vi "beepstatus.vi"() -> ()   [LabVIEW 2026]
panel:
  in  "running":bool
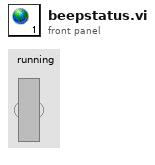
[diagram p1: front panel]
diagram:
